vi "modify channel test.vi"() -> (0 "no err":errorcluster, 3 "mod success":bool)   [LabVIEW 2015, in "DAQmx Module Tests.lvlib"]
doc: "Tests the 'Replace Line' VI."
uses:
  DAQmx Module Tests.lvlib
  <vilib>/NI/Tag Bus Module Framework/channel/TBM channel.lvclass/TBM channel.ctl
  <vilib>/NI/Tag Bus Module Framework/channel/channel classification.ctl
  <vilib>/NI/Tag Bus/tag/tag descriptor.lvclass/tag descriptor.ctl
  <vilib>/NI/Tag Bus Module Framework/channel/Read channel classification.vi
  <vilib>/NI/Tag Bus Module Framework/channel/Write channel classification.vi
  module/configuration/Daqmx Module configuration.lvclass
  <vilib>/NI/Tag Bus Module Framework/channel/TBM channel.lvclass
  <vilib>/NI/Tag Bus/tag/tag descriptor.lvclass
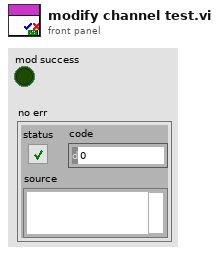
[diagram p1: front panel]
types:
  T1 = typedef "DAQmx Module Configuration.lvclass/Line.ctl" = cluster{"Channel Array":refnum<class "TBM channel.lvclass">[], "Physical Channel":string, "Measurement Type":T2, "Parameters":T3}
  T2 = typedef "DAQmx Module Configuration.lvclass/Measurement Type.ctl" = enum16{"Digital Input", "Digital Output", "Voltage Input", "Voltage Output", "Current Input", "Current Output", "RTD", "Thermocouple", "Strain", "PWM"}
  T3 = typedef "DAQmx Module Configuration.lvclass/Parameters.ctl" = cluster{"Digital Config":cluster{"Invert Lines?":bool}, "Voltage Config":cluster{"Maximum Value (V)":dbl, "Minimum Value (V)":dbl, "in terminal configuration (V)":i32, "out terminal configuration (V)":i32}, "Current Config":cluster{"Maximum Value (A)":dbl, "Minimum Value (A)":dbl, "shunt resistor location":i32, "input terminal configuration (C)":i32, "external shunt resistor value":dbl}, "RTD Config":cluster{"Maximum Value (°C)":dbl, "Minimum Value (°C)":dbl, "resistance configuration":i32, "r0":dbl, "current excitation value":dbl, "rtd type":i32, "current excitation source":i32}, "Thermocouple Config":cluster{"Minimum Value (C)":dbl, "Maximum Value (C)":dbl, "thermocouple type":i32, "cjc source":i32, "cjc value":dbl}, "Strain Config":cluster{"Maximum Value":dbl, "Minimum Value":dbl, "bridge information":cluster{"strain configuration":i32, "lead wire resistance":dbl, "initial bridge voltage":dbl, "voltage excitation source":i32, "voltage excitation value":dbl}, "strain gage information":cluster{"gage factor":dbl, "nominal gage resistance":dbl, "poisson ratio":dbl}}, "PWM Config":cluster{"Idle State":bool}}
  T4 = typedef "TBM channel.lvclass/channel classification.ctl" = enum16{"input data", "output data", "processing parameter", "processing result"}
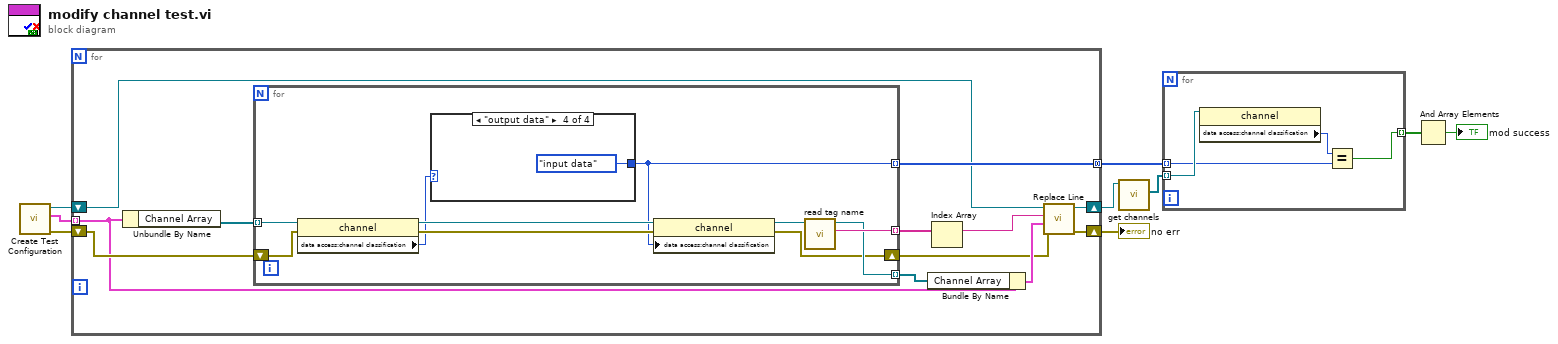
[diagram p0: block diagram]
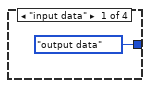
[diagram p2: hidden frame]
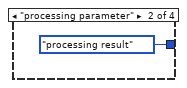
[diagram p3: hidden frame]
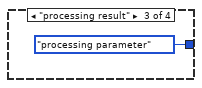
[diagram p4: hidden frame]
diagram:
  n1 = call "Create Test Configuration.vi"() -> ("error out"=w1:errorcluster, "Line Array"=w2:T1[], "Module Configuration"=w3:refnum<class "Daqmx Module configuration.lvclass">)  [unwired: 6 in, 3 out]
  n2 = for {
    shift-right: [w17] -> w9
    shift-left: w3 -> [w16]
    shift-right: [w18] -> w8
    shift-left: w1 -> [w21]
    tunnel: w2 -> [w15] mode=indexing
    tunnel: [w20] -> w4 mode=concatenating
    n3 = Unbundle By Name(w15) -> ("Channel Array"=w19:refnum<class "TBM channel.lvclass">[])
    n4 = for {
      tunnel: [w27] -> w20 mode=indexing
      tunnel: w19 -> [w26] mode=indexing
      tunnel: [w25] -> w13 mode=indexing
      tunnel: [w23] -> w12 mode=indexing
      shift-right: [w22] -> w11
      shift-left: w21 -> [w31]
      n5 = property class="channel"(reference=w26, error in=w31) -> (reference out=w29:refnum<class "TBM channel.lvclass">, error out=w30:errorcluster, "data access:channel classification"=w28:T4)
      n6 = case shown="\"output data\"" w28 {
        tunnel: [channel_classification."output data" ("channel classification") channel_classification."processing result" ("channel classification") channel_classification."processing parameter" ("channel classification") channel_classification."input data" ("channel classification")] -> w27
        frame "input data" {
        }
        frame "processing parameter" {
        }
        frame "processing result" {
        }
        frame "output data" {
        }
      }
      n7 = property class="channel"(reference=w29, error in=w30, "data access:channel classification"=w27) -> (reference out=w24:refnum<class "TBM channel.lvclass">, error out=w22:errorcluster)
      n8 = call <vilib>:"read tag name.vi"("system tag in"=w24) -> ("name"=w25:string, "system tag out"=w23:refnum<class "TBM channel.lvclass">)  [unwired: 8 in, 1 out]
    }
    n9 = Bundle By Name(cluster=w15, "Channel Array"=w12) -> (w14:T1)
    n10 = Index Array(array=w13) -> (element=w10:string)  [unwired: 1 in]
    n11 = call "Replace Line.vi"("error in"=w11, "New Line"=w14, "Line Name"=w10, "Daqmx Module configuration in"=w16) -> ("error out"=w18:errorcluster, "Daqmx Module configuration out"=w17:refnum<class "Daqmx Module configuration.lvclass">)  [unwired: 5 in, 1 out]
  }
  "no err" <- w8
  n12 = call-dynamic "get channels.vi"("Daqmx Module configuration in"=w9) -> ("channels"=w7:refnum<class "TBM channel.lvclass">[])  [unwired: 9 in, 1 out]
  n13 = for {
    tunnel: w7 -> [w39] mode=indexing
    tunnel: [w36] -> w6 mode=indexing
    tunnel: w4 -> [w38] mode=indexing
    n14 = property class="channel"(reference=w39) -> ("data access:channel classification"=w37:T4)  [unwired: 1 in, 2 out]
    n15 = Equal?(x=w37, y=w38) -> (x = y?=w36:bool)
  }
  n16 = And Array Elements(Boolean array=w6) -> (logical AND=→"mod success":bool)
